vi "Is Index In Range (2D Array).vi"(1 "Column Index":i32, 2 "Row Index":i32, 3 "2D Array Sizes":i32[](array[numeric])) -> (0 "Are Both Indexes In Range?":bool)   [LabVIEW 2026, in "RSysUtils Array.lvlib"]
doc: "This VI checks whether a pair of row and column indexes point to a valid element of a 2D array."
uses:
  RSysUtils Array.lvlib
panel:
  out "2D Array Number of Columns":i32
  out "2D Array Number of Rows":i32
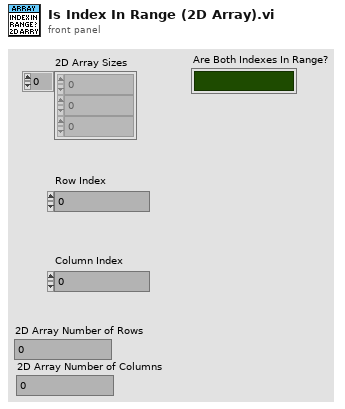
[diagram p1: front panel]
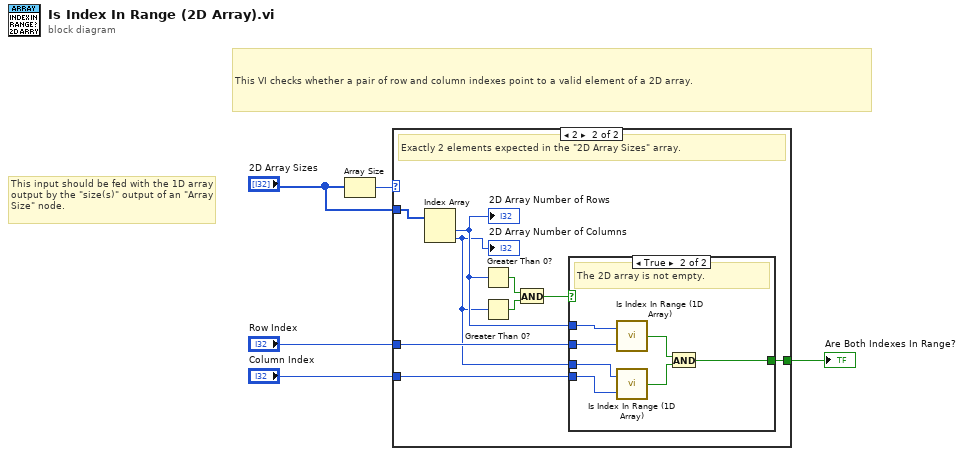
[diagram p0: block diagram]
diagram:
  # "This input should be fed with the 1D array output by the \"size(s)\" output of an \"Array Size\" node."
  # "This VI checks whether a pair of row and column indexes point to a valid element of a 2D array."
  n1 = Array Size(array="2D Array Sizes") -> (size(s)=w5:i32)
  n2 = case shown="2" w5 {
    tunnel: "2D Array Sizes" -> [_ w14]
    tunnel: "Row Index" -> [_ w10]
    tunnel: "Column Index" -> [_ w9]
    tunnel: [_ w6] -> w1
    frame Default {
      # "Unexpected number of sizes"
    }
    frame 2 {
      # "Exactly 2 elements expected in the \"2D Array Sizes\" array."
      n3 = Index Array(array=w14) -> (element #1=w8:i32, element #2=w7:i32)  [unwired: 2 in]
      "2D Array Number of Rows" <- w8
      "2D Array Number of Columns" <- w7
      n4 = Greater Than 0?(x=w8) -> (x > 0?=w13:bool)
      n5 = Greater Than 0?(x=w7) -> (x > 0?=w12:bool)
      n6 = And(x=w13, y=w12) -> (x .and. y?=w11:bool)
      n7 = case shown="True" w11 {
        tunnel: w10 -> [_ w20]
        tunnel: w9 -> [_ w18]
        tunnel: w8 -> [_ w21]
        tunnel: w7 -> [_ w19]
        tunnel: [_ w15] -> w6
        frame False {
          # "The 2D array is empty."
        }
        frame True {
          # "The 2D array is not empty."
          n8 = call "Is Index In Range (1D Array).vi"("Index"=w20, "Array Number of Elements (Array Size)"=w21) -> ("Is Index In Range?"=w16:bool)
          n9 = call "Is Index In Range (1D Array).vi"("Index"=w18, "Array Number of Elements (Array Size)"=w19) -> ("Is Index In Range?"=w17:bool)
          n10 = And(x=w16, y=w17) -> (x .and. y?=w15:bool)
        }
      }
    }
  }
  "Are Both Indexes In Range?" <- w1
